vi "Exo_sequence.vi"() -> ()   [LabVIEW 2012]
panel:
  out "M":dbl
  in  "B":dbl
  in  "A":dbl
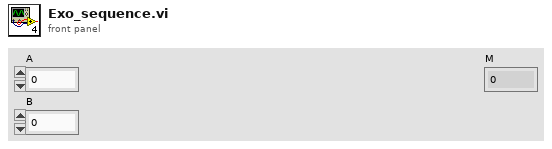
[diagram p1: front panel]
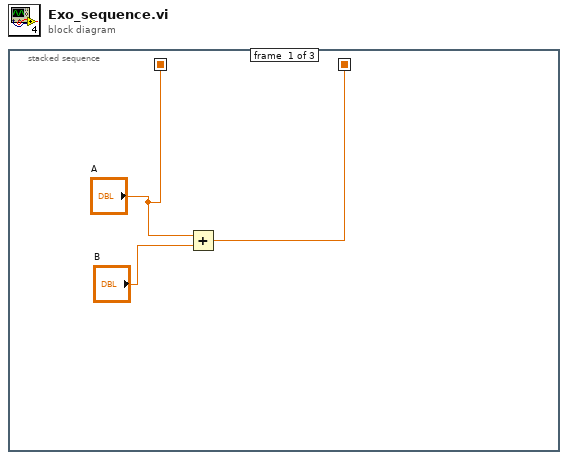
[diagram p0: block diagram]
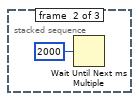
[diagram p2: hidden frame]
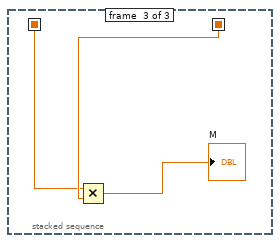
[diagram p3: hidden frame]
diagram:
  n1 = stacked-sequence {
    seq-local: [w2 _ _] -> [_ _ w7]
    seq-local: ["A" _ _] -> [_ _ w5]
    frame #0 {
      n2 = Add(x="A", y="B") -> (x+y=w2:dbl)
    }
    frame #1 {
      n3 = Wait Until Next ms Multiple(millisecond multiple=u32 2000) -> ()  [unwired: 1 out]
    }
    frame #2 {
      n4 = Multiply(x=w5, y=w7) -> (x*y=→"M":dbl)
    }
  }
